vi "property.get.vi"   [LabVIEW 2020, in "asset.lvclass"]
uses:
  asset.lvclass
  asset.lvclass/asset.ctl
  attachments.get.vi
  createdAt.get.vi
  createdBy.get.vi
  datascopes.get.vi
  description.get.vi
  isArchived.get.vi
  isStaged.get.vi
  labels.get.vi
  links.get.vi
  properties.get.vi
  rid.get.vi
  type.get.vi
  updatedAt.get.vi
  nominal types/labels/to_array.vi
  nominal types/labels/labels.get.vi
  nominal types/properties/to.cluster_pairs.vi
  title.get.vi
  Nominal Client/type.get.vi
  nominal types/labels/labels.lvclass
  nominal types/properties/properties.lvclass
  type/type.lvclass
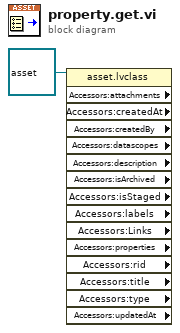
[diagram p0: block diagram]
diagram:
  n1 = property class="asset.lvclass" props=["Accessors:attachments", "Accessors:createdAt", "Accessors:createdBy", "Accessors:datascopes", "Accessors:description", "Accessors:isArchived", "Accessors:isStaged", "Accessors:labels", "Accessors:Links", "Accessors:properties", "Accessors:rid", "Accessors:title", "Accessors:type", "Accessors:updatedAt"](reference=refnum<class "asset.lvclass"> refnum ("asset.lvclass")) -> ()  [unwired: 1 in, 16 out]
